vi "Plot Multi-XY.vi"(0 "picture":picture, 1 "desired font(Application)":T5(ring)=enum."Application Font", 2 "Draw Axes":bool, 3 "[user-specified font]":T6, 5 "data":cluster{"data":cluster{"x":dbl, "y":dbl}[]}[](array[cluster]) {"data"."y" format="%0.2f"; "data"."x" format="%0.2f"}, 7 "dimensions (w,h)":cluster{"width":i16, "height":i16}, 11 "top left point(0, 0)":cluster{"x":i16, "y":i16}, 12 "cartesian axis attributes":T7={"x minimum"=0.0, "x maximum"=0.0, "x log?"=FALSE, "x precision"=1, "x format"=enum."Decimal", "y minimum"=0.0, "y maximum"=0.0, "y log?"=FALSE, "y precision"=1, "y format"=enum."Decimal"} {"x minimum" format="%0.2f"; "x maximum" format="%0.2f"; "y minimum" format="%0.2f"; "y maximum" format="%0.2f"}, 13 "cartesian grid cosmetics":T2={"line color"=39168, "text color"=65280, "tick length(3)"=3, "crossing axes"=FALSE, "visible grid?"=TRUE}, 14 "XY plot cosmetics":T4(array[cluster])=[{"plot color"=16776960, "XY plot type"=enum."sized scatter plot", "baseline"=0.0}, {"plot color"=65280, "XY plot type"=enum."connected points", "baseline"=0.0}, {"plot color"=65535, "XY plot type"=enum."connected points", "baseline"=0.0}] {"baseline" format="%0.2f"}, 15 "[sized scatter plot cosmetics]":T1(array[cluster])=[{"min size"=1, "max size"=5, "maps to max size"=5, "color array"=[16776960, 65280, 16711680, 255]}]) -> (4 "new picture":picture)   [LabVIEW 2012, in "Vector Function Generator.xctl"]
doc: "Takes a picture and an array of plots and appends a picture of an XY graph of the data with the plots overlaid on the same graph. Original version modified by G. Burnell (g.burnell@leeds.ac.uk) for plotting on black background."
uses:
  Vector Function Generator.xctl
  <vilib>/picture/cartesn2.llb/XY Plot Type.ctl
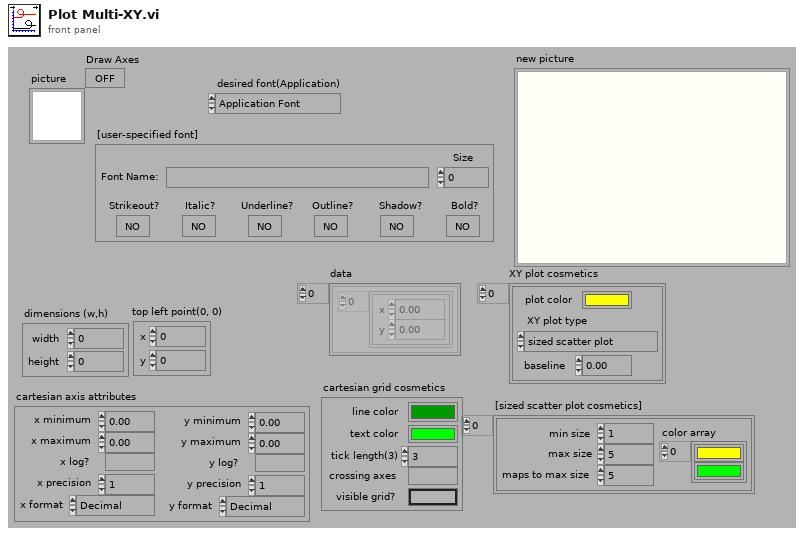
[diagram p1: front panel]
types:
  T1 = cluster{"min size":i16, "max size":i16, "maps to max size":i16, "color array":u32[]}[]
  T2 = cluster{"line color":u32, "text color":u32, "tick length(3)":i16, "crossing axes":bool, "visible grid?":bool}
  T3 = typedef "XY Plot Type.ctl" = enum16{"points", "squares", "circles", "connected points", "connected squares", "connected circles", "comb plot", "sized scatter plot", "sized-colored scatter plot", "min-max lines"}
  T4 = cluster{"plot color":u32, "XY plot type":T3, "baseline":dbl}[]
  T5 = enum16{"User-specified Font", "Application Font", "System Font", "Dialog Font"}
  T6 = cluster{"Font Name:":string, "Size":i16, "Strikeout?":bool, "Italic?":bool, "Underline?":bool, "Outline?":bool, "Shadow?":bool, "Bold?":bool}
  T7 = cluster{"x minimum":dbl, "x maximum":dbl, "x log?":bool, "x precision":u8, "x format":enum8{"Decimal", "Scientific", "Engineering", "Binary", "Octal", "Hex"}, "y minimum":dbl, "y maximum":dbl, "y log?":bool, "y precision":u8, "y format":enum8{"Decimal", "Scientific", "Engineering", "Binary", "Octal", "Hex"}}
  T8 = cluster{"left":i16, "top":i16, "right":i16, "bottom":i16}
  T9 = cluster{"plot color":u32, "XY plot type":T3, "baseline":dbl}
  T10 = cluster{"min size":i16, "max size":i16, "maps to max size":i16, "color array":u32[]}
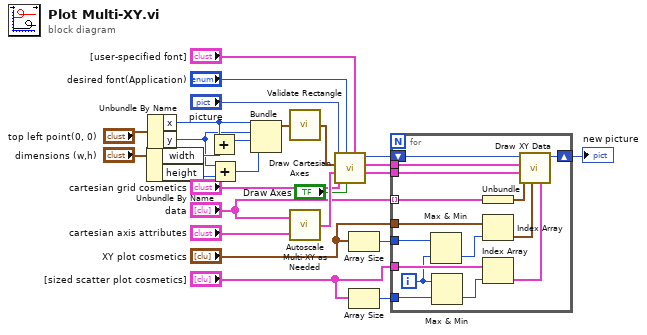
[diagram p0: block diagram]
diagram:
  n1 = Unbundle By Name("dimensions (w,h)") -> ("width"=w10:i16, "height"=w9:i16)
  n2 = Unbundle By Name("top left point(0, 0)") -> ("x"=w8:i16, "y"=w7:i16)
  n3 = Add(x=w8, y=w10) -> (x+y=w6:i16)
  n4 = Add(x=w7, y=w9) -> (x+y=w5:i16)
  n5 = Bundle("x"=w8, "y"=w7, w6, w5) -> (w2:cluster{"x":i16, "y":i16, i16, i16})  [unwired: 1 out]
  n6 = call <vilib>:"Validate Rectangle.vi"("rect"=w2) -> ("valid rect"=w18:T8)
  n7 = call <vilib>:"Autoscale Multi-XY as Needed.vi"("axis attributes"="cartesian axis attributes", "multi-xy data"="data") -> ("axis attributes"=w26:T7)
  n8 = call "Draw Cartesian Axes.vi"("[user-specified font]"="[user-specified font]", "Draw Axes"="Draw Axes", "desired font(Application)"="desired font(Application)", "grid cosmetics"="cartesian grid cosmetics", "axis attributes"=w26, "bounding rect"=w18, "picture"="picture") -> ("y scale factors"=w19:cluster{"a":dbl, "b":dbl, "log?":bool}, "x scale factors"=w20:cluster{"a":dbl, "b":dbl, "log?":bool}, "new picture"=w23:picture)  [unwired: 2 out]
  n9 = Array Size(array="XY plot cosmetics") -> (size(s)=w11:i32)
  n10 = Array Size(array="[sized scatter plot cosmetics]") -> (size(s)=w13:i32)
  n11 = for {
    shift-right: [w38] -> w22
    shift-left: w23 -> [w39]
    tunnel: w19 -> [w41]
    tunnel: w20 -> [w40]
    tunnel: "XY plot cosmetics" -> [w37]
    tunnel: "data" -> [w36] mode=indexing
    tunnel: "[sized scatter plot cosmetics]" -> [w33]
    tunnel: w13 -> [w31]
    tunnel: w11 -> [w28]
    i -> [w27]
    n12 = Max & Min(x=w28, y=w27) -> (min(x,y)=w29:i32)  [unwired: 1 out]
    n13 = Max & Min(x=w27, y=w31) -> (min(x,y)=w30:i32)  [unwired: 1 out]
    n14 = Unbundle(w36) -> ("data"=w35:cluster{"x":dbl, "y":dbl}[])
    n15 = Index Array(array=w37, index=w29) -> (element=w34:T9)
    n16 = Index Array(array=w33, index=w30) -> (element=w32:T10)
    n17 = call "Draw XY Data.vi"("[sized scatter plot cosmetics]"=w32, "xy cosmetics"=w34, "xy data"=w35, "y scale factors"=w41, "x scale factors"=w40, "picture"=w39) -> ("new picture"=w38:picture)  [unwired: 5 out]
  }
  "new picture" <- w22
